vi "to_table.vi"(8 "error in (no error)":errorcluster, 11 "Item in":refnum<class "Item.lvclass">) -> (0 "error out":errorcluster, 3 "Table":refnum<class "Table.lvclass">)   [LabVIEW 2020, in "toml_edit.lvlib" / "Item.lvclass"]
uses:
  Item.lvclass
  Table/Table.lvclass
  Item.lvclass/Item.ctl
  type--enum.ctl
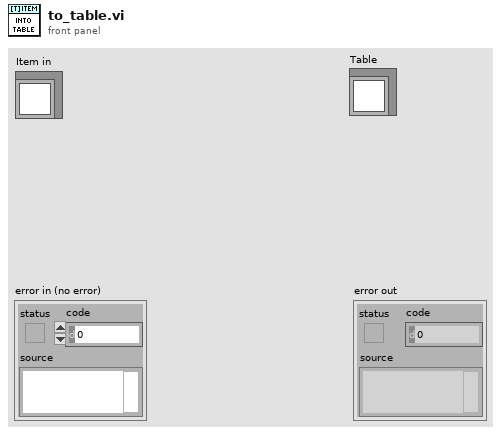
[diagram p1: front panel]
types:
  T1 = typedef "toml_edit.lvlib/Item.lvclass/type--enum.ctl" = enum16{"Unknown", "None", "Value", "ArrayOfTables", "Table"}
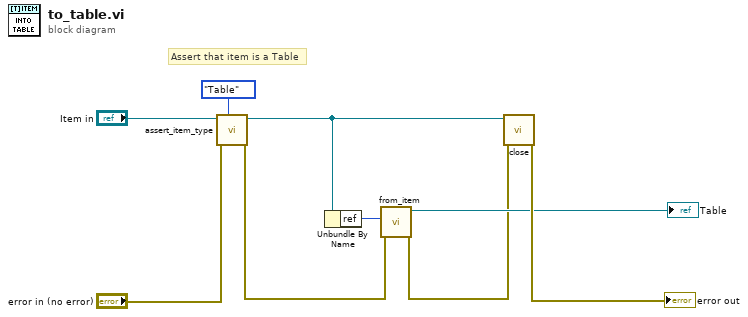
[diagram p0: block diagram]
diagram:
  # "Assert that item is a Table"
  n1 = call "assert_item_type.vi"("item_type"=type--enum."Table", "error in (no error)"="error in (no error)", "Item in"="Item in") -> ("error out"=w3:errorcluster, "Item out"=w4:refnum<class "Item.lvclass">)  [unwired: 7 in]
  n2 = Unbundle By Name(w4) -> ("ref"=w6:u64)
  n3 = call "from_item.vi"("error in (no error)"=w3, "item_ref"=w6) -> ("error out"=w2:errorcluster, "Table out"=→"Table":refnum<class "Table.lvclass">)  [unwired: 8 in]
  n4 = call "close.vi"("error in (no error)"=w2, "Item in"=w4) -> ("error out"=→"error out":errorcluster)  [unwired: 9 in]
